vi "Get Engine from HAL.vi"(8 "error in (no error)":errorcluster, 9 "Instrument":string, 10 "Engine":string, 11 "XY Plotter in":refnum<class "XY Plotter.lvclass">) -> (0 "error out":errorcluster, 1 "Waveforms":waveform(dbl)[](array[waveform]), 2 "Channels":string[](array[string]), 3 "XY Plotter out":refnum<class "XY Plotter.lvclass">)   [LabVIEW 2025, in "XY Plotter.lvlib" / "XY Plotter.lvclass"]
uses:
  XY Plotter.lvclass
  C:/Users/Public/Documents/Sandia National Labs/TSS Plugin/CEF.lvlibp/Node/CEF_Node.lvclass
  Users/Public/Documents/Sandia National Labs/TSS Plugin/Abstract.lvlibp/Abstract Engine/Abstract Engine.lvclass
  Users/Public/Documents/Sandia National Labs/TSS Plugin/Abstract.lvlibp/Abstract Instrument/Abstract Instrument.lvclass
  Users/Public/Documents/Sandia National Labs/TSS Plugin/CEF.lvlibp/Node/ReadParent.vi
  Users/Public/Documents/Sandia National Labs/TSS Plugin/CEF.lvlibp/Node/ReadChildren.vi
  Users/Public/Documents/Sandia National Labs/TSS Plugin/Abstract.lvlibp/Abstract Engine/Read Engine Cluster.vi
  Users/Public/Documents/Sandia National Labs/TSS Plugin/CEF.lvlibp/Node/CEF_Node.lvclass
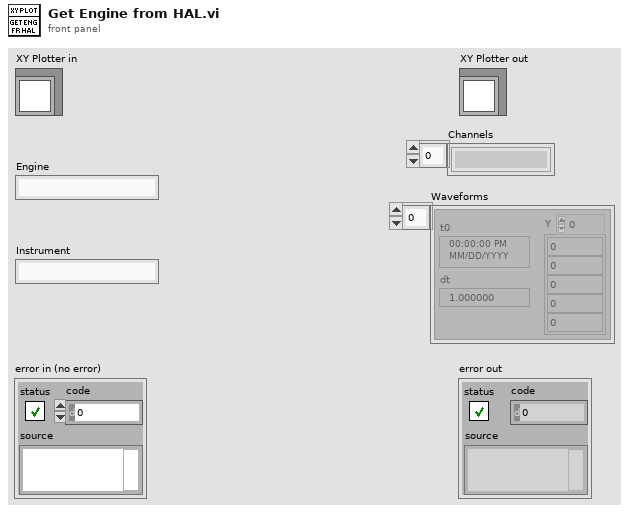
[diagram p1: front panel]
types:
  T1 = typedef "Abstract.lvlibp/Abstract Engine.lvclass/Engine Cluster.ctl" = cluster{"Initialized":bool, "IP Address":string, "Engine Type":string, "InstrumentMap":map{string, cluster{"Initialized":bool, "IP Address":string, "Instr Type":string, "Channels":cluster{"Enable":bool, "Alias":string}[]}}}
  T2 = map{string, cluster{"Initialized":bool, "IP Address":string, "Instr Type":string, "Channels":cluster{"Enable":bool, "Alias":string}[]}}
  T3 = cluster{"Initialized":bool, "IP Address":string, "Instr Type":string, "Channels":cluster{"Enable":bool, "Alias":string}[]}
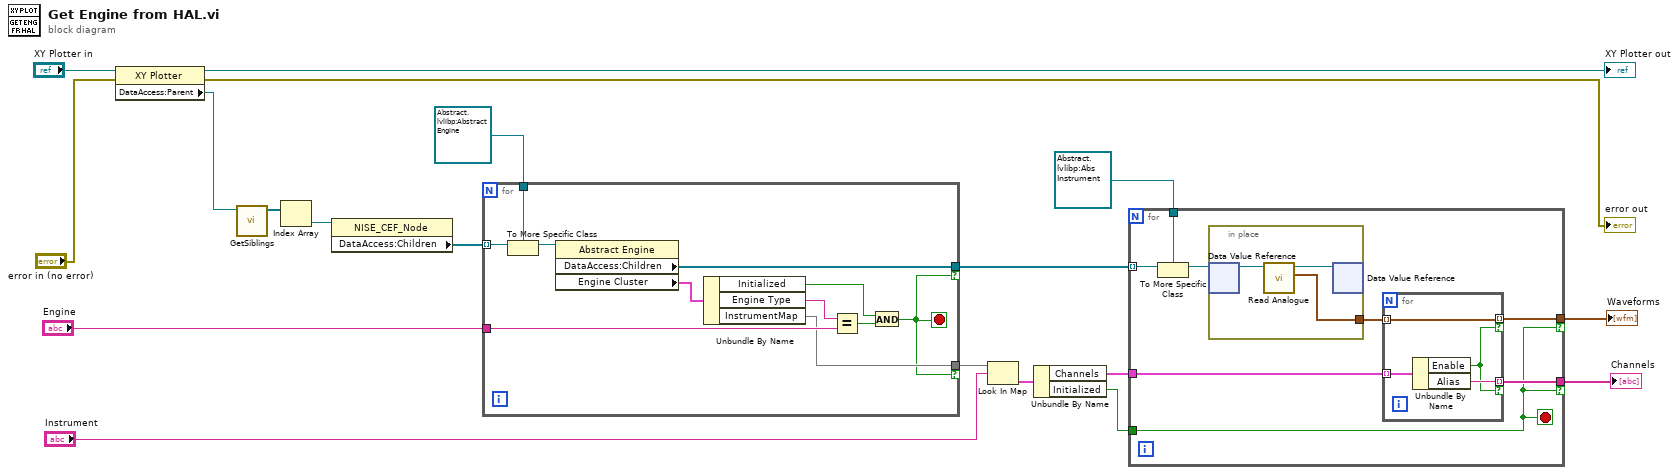
[diagram p0: block diagram]
diagram:
  n1 = property class="XY Plotter"(reference="XY Plotter in", error in="error in (no error)") -> (reference out=→"XY Plotter out":refnum<class "XY Plotter.lvclass">, error out=→"error out":errorcluster, "DataAccess:Parent"=w16:refnum<data-value>)
  n2 = call "GetSiblings.vi"("node in"=w16) -> ("siblings"=w15:refnum<data-value>[])  [unwired: 9 in, 1 out]
  n3 = Index Array(array=w15) -> (element=w14:refnum<data-value>)  [unwired: 1 in]
  n4 = property class="NISE_CEF_Node"(reference=w14) -> ("DataAccess:Children"=w13:refnum<data-value>[])  [unwired: 1 in, 2 out]
  n5 = for {
    tunnel: w13 -> [w30] mode=indexing
    tunnel: refnum<data-value> refnum ("data value reference") -> [w29]
    tunnel: "Engine" -> [w26]
    tunnel: [w22] -> w9 if=w20
    tunnel: [w21] -> w6 if=w20
    stop <- w20 stop-if-true
    n6 = To More Specific Class(target class=w29, reference=w30) -> (specific class reference=w28:refnum<data-value>)  [unwired: 1 in, 1 out]
    n7 = property class="Abstract Engine"(reference=w28) -> ("DataAccess:Children"=w22:refnum<data-value>[], "Engine Cluster"=w23:T1)  [unwired: 1 in, 2 out]
    n8 = Unbundle By Name(w23) -> ("Initialized"=w25:bool, "Engine Type"=w27:string, "InstrumentMap"=w21:T2)
    n9 = Equal?(x=w27, y=w26) -> (x = y?=w24:bool)
    n10 = And(x=w25, y=w24) -> (x .and. y?=w20:bool)
  }
  n11 = Look In Map(map=w6, key="Instrument") -> (value=w4:T3)  [unwired: 1 in, 1 out]
  n12 = Unbundle By Name(w4) -> ("Channels"=w3:cluster{"Enable":bool, "Alias":string}[], "Initialized"=w2:bool)
  n13 = for {
    tunnel: w9 -> [w38] mode=indexing
    tunnel: refnum<data-value> refnum ("data value reference") -> [w37]
    tunnel: [w33] -> w7 if=w31
    tunnel: w2 -> [w31]
    tunnel: w3 -> [w35]
    tunnel: [w32] -> w1 if=w31
    stop <- w31 stop-if-true
    n14 = To More Specific Class(target class=w37, reference=w38) -> (specific class reference=w36:refnum<data-value>)  [unwired: 1 in, 1 out]
    n15 = in-place {
      in-place-border: [w39] -> w34
      n16 = in-place-dvr #1(w36) -> (w41:refnum<class "Abstract Instrument.lvclass">)  [unwired: 1 out]
      n17 = call-dynamic "Read Analogue.vi"("Analog Input in"=w41) -> ("Waveforms"=w39:waveform(dbl)[], "Analog Input out"=w40:refnum<class "Abstract Instrument.lvclass">)  [unwired: 8 in, 1 out]
      n18 = in-place-dvr #1(w40) -> ()  [unwired: 2 out]
    }
    n19 = for {
      tunnel: w35 -> [w45] mode=indexing
      tunnel: w34 -> [w44] mode=indexing
      tunnel: [w44] -> w33 mode=indexing if=w42
      tunnel: [w43] -> w32 mode=indexing if=w42
      n20 = Unbundle By Name(w45) -> ("Enable"=w42:bool, "Alias"=w43:string)
    }
  }
  "Waveforms" <- w7
  "Channels" <- w1
